vi "createSelfReference.vi"(8 "error in (no error)":errorcluster, 11 "Connection in":refnum<class "Connection.lvclass">) -> (0 "error out":errorcluster, 3 "Connection out":refnum<class "Connection.lvclass">)   [LabVIEW 2013, in "Connection_GOSPL.lvlib" / "Connection.lvclass"]
uses:
  Connection.lvclass
  connection event -- cluster.ctl
  Connection.lvclass/Connection.ctl
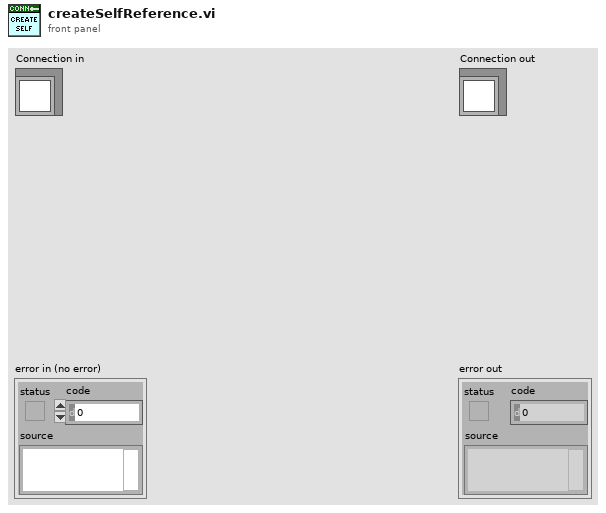
[diagram p1: front panel]
types:
  T1 = typedef "Connection_GOSPL.lvlib/Connection.lvclass/connection event -- cluster.ctl" = cluster{"connected":bool, "reason":i32}
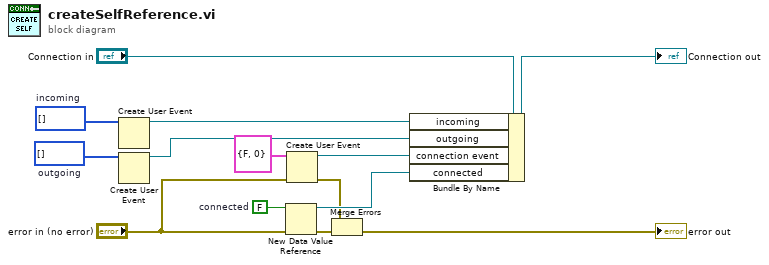
[diagram p0: block diagram]
diagram:
  w3 = u8[] []  # outgoing
  w4 = u8[] []  # incoming
  w12 = FALSE  # connected
  n1 = Create User Event(user event datatype=w4) -> (user event=w2:refnum<user-event>)  [unwired: 1 in, 1 out]
  n2 = Create User Event(user event datatype=w3) -> (user event=w1:refnum<user-event>)  [unwired: 1 in, 1 out]
  n3 = New Data Value Reference(data value=w12, error in="error in (no error)") -> (data value reference=w11:refnum<data-value>, error out=w6:errorcluster)
  n4 = Create User Event(user event datatype=T1 {"connected"=FALSE, "reason"=0} ("Connection event"), error in="error in (no error)") -> (user event=w9:refnum<user-event>, error out=w7:errorcluster)
  n5 = Merge Errors(w7, w6) -> (→"error out":errorcluster)
  n6 = Bundle By Name(cluster="Connection in", "incoming"=w2, "outgoing"=w1, "connection event"=w9, "connected"=w11) -> (→"Connection out":refnum<class "Connection.lvclass">)
